vi "RemoteVI Fixture Log Path.vi"(0 "Log Path":path, 11 "error in":errorcluster) -> (4 "path":path, 15 "error out":errorcluster)   [LabVIEW 2020]
doc: "Event-log helper of RemoteVI Fixture.vi. Returns Log Path, or RemoteVI Fixture.log in the system temp directory when Log Path is empty. error in is passed through unchanged."
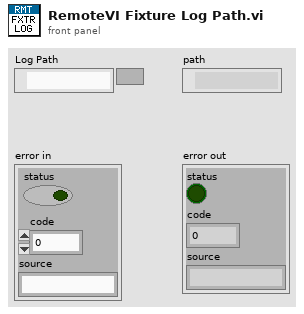
[diagram p1: front panel]
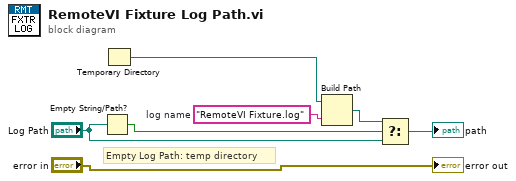
[diagram p0: block diagram]
diagram:
  w5 = "RemoteVI Fixture.log"  # log name
  # "Empty Log Path: temp directory"
  n1 = Empty String/Path?(string/path="Log Path") -> (empty?=w3:bool)
  n2 = Temporary Directory() -> (w4:path)
  n3 = Build Path(base path=w4, name or relative path=w5) -> (appended path=w6:path)
  n4 = Select(t=w6, s=w3, f="Log Path") -> (s? t:f=→"path":path)
  "error out" <- "error in"
